vi "measure BT Audio Frequency Separation Step3.vi"(8 "error in (no error)":errorcluster, 11 "SA Measurement in":refnum<class "SA Measurement.lvclass">) -> (0 "error out":errorcluster, 3 "SA Measurement out":refnum<class "SA Measurement.lvclass">)   [LabVIEW 2023, in "Spectrum Analyzer.lvlib" / "SA Measurement.lvclass"]
uses:
  SA Measurement.lvclass
  SA Measurement.lvclass/SA Measurement.ctl
  Interface_Spectrum/Interface_Spectrum.lvclass
  TYPE DEFINITION/TYPE Marker Control Mode.ctl
  Spectrum Analyzer.lvlib
  TYPE DEFINITION/TYPE Marker Peak Search Type.ctl
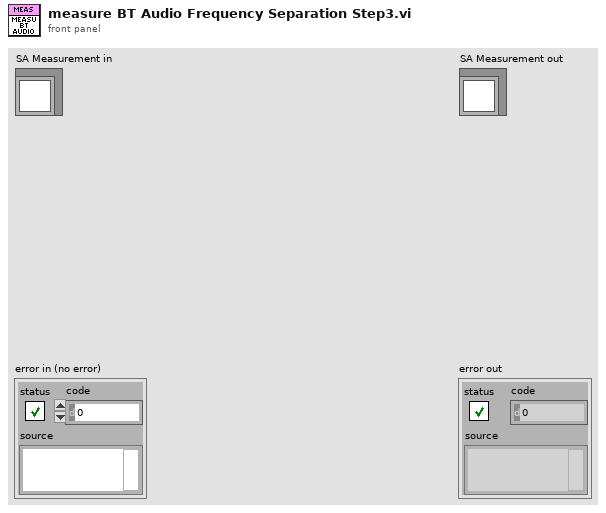
[diagram p1: front panel]
types:
  T1 = typedef "Spectrum Analyzer.lvlib/TYPE Marker Control Mode.ctl" = enum16{"Normal", "Delta", "Off"}
  T2 = typedef "Spectrum Analyzer.lvlib/TYPE Marker Peak Search Type.ctl" = enum16{"Max", "Next Peak"}
  T3 = typedef "Spectrum Analyzer.lvlib/TYPE Marker Value.ctl" = cluster{"X-axis":dbl, "Y-axis":dbl}
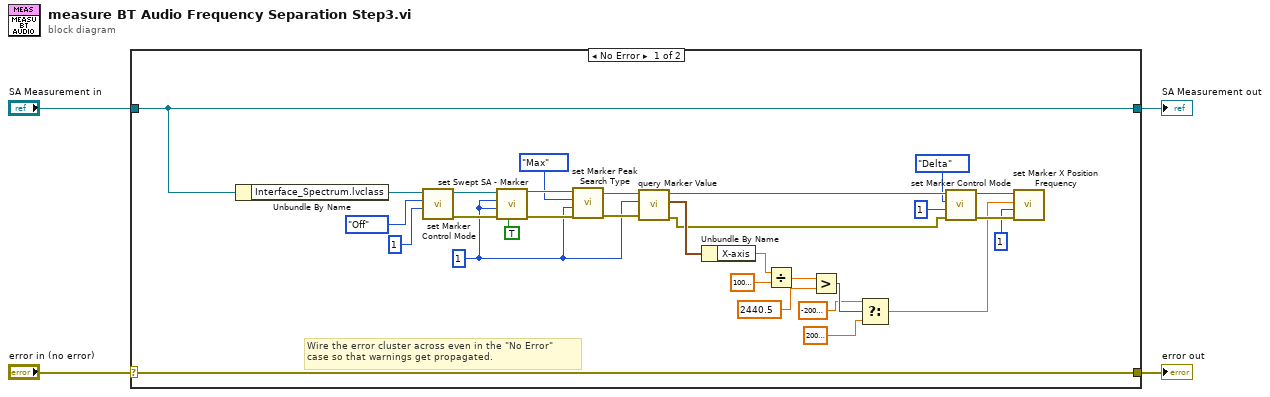
[diagram p0: block diagram]
diagram:
  n1 = case shown="No Error" "error in (no error)" {
    selector: "error in (no error)" -> [w34 w36]
    tunnel: [w34 w36] -> w3
    tunnel: [w33 w35] -> w1
    tunnel: "SA Measurement in" -> [w33 w35]
    frame No Error {
      w21 = 1 ("Index")
      # "Wire the error cluster across even in the \"No Error\"\ncase so that warnings get propagated."
      n2 = Unbundle By Name(w33) -> ("Interface_Spectrum.lvclass"=w32:refnum<class "Interface_Spectrum.lvclass">)
      n3 = call-dynamic "set Marker Control Mode.vi"("Marker Index"=1, "Marker Mode"=TYPE_Marker_Control_Mode."Off", "Interface_Spectrum in"=w32) -> ("error out"=w24:errorcluster, "Interface_Spectrum out"=w25:refnum<class "Interface_Spectrum.lvclass">)  [unwired: 7 in]
      n4 = call-dynamic "set Swept SA - Marker.vi"("On?"=TRUE, "error in (no error)"=w24, "trace"=w21, "Index"=w21, "Interface_Spectrum in"=w25) -> ("error out"=w27:errorcluster, "Interface_Spectrum out"=w28:refnum<class "Interface_Spectrum.lvclass">)  [unwired: 5 in]
      n5 = call-dynamic "set Marker Peak Search Type.vi"("error in (no error)"=w27, "Marker Index"=w21, "Peak Search Type"=TYPE_Marker_Peak_Search_Type."Max", "Interface_Spectrum in"=w28) -> ("error out"=w22:errorcluster, "Interface_Spectrum out"=w23:refnum<class "Interface_Spectrum.lvclass">)  [unwired: 6 in]
      n6 = call-dynamic "query Marker Value.vi"("error in (no error)"=w22, "Marker Index"=w21, "Interface_Spectrum in"=w23) -> ("error out"=w9:errorcluster, "Marker Value"=w20:T3, "Interface_Spectrum out"=w12:refnum<class "Interface_Spectrum.lvclass">)  [unwired: 6 in]
      n7 = Unbundle By Name(w20) -> ("X-axis"=w13:dbl)
      n8 = Divide(x=w13, y=1000000.0) -> (x/y=w18:dbl)
      n9 = Greater?(x=w18, y=2440.5) -> (0:w16:bool)
      n10 = Select(t=-2000000.0 ("Value"), s=w16, f=2000000.0 ("Value")) -> (s? t:f=w5:dbl)
      n11 = call-dynamic "set Marker Control Mode.vi"("error in (no error)"=w9, "Marker Index"=1, "Marker Mode"=TYPE_Marker_Control_Mode."Delta", "Interface_Spectrum in"=w12) -> ("error out"=w7:errorcluster, "Interface_Spectrum out"=w8:refnum<class "Interface_Spectrum.lvclass">)  [unwired: 6 in]
      n12 = call-dynamic "set Marker X Position Frequency.vi"("error in (no error)"=w7, "Index"=1, "X Position Frequency (Hz)"=w5, "Interface_Spectrum in"=w8) -> ()  [unwired: 6 in, 2 out]
    }
    frame Error {
    }
  }
  "error out" <- w3
  "SA Measurement out" <- w1
